vi "turn on off Keysight 9020A Correction Factor.vi"(8 "error in (no error)":errorcluster, 9 "Correction Applied?":bool, 10 "Target Correction Table":T1(ring), 11 "Keysight 9020A in":refnum<class "Keysight 9020A.lvclass">) -> (0 "error out":errorcluster, 3 "Keysight 9020A out":refnum<class "Keysight 9020A.lvclass">)   [LabVIEW 2023, in "Spectrum Analyzer.lvlib" / "Keysight 9020A.lvclass"]
uses:
  Keysight 9020A.lvclass
  Keysight 9020A.lvclass/Keysight 9020A.ctl
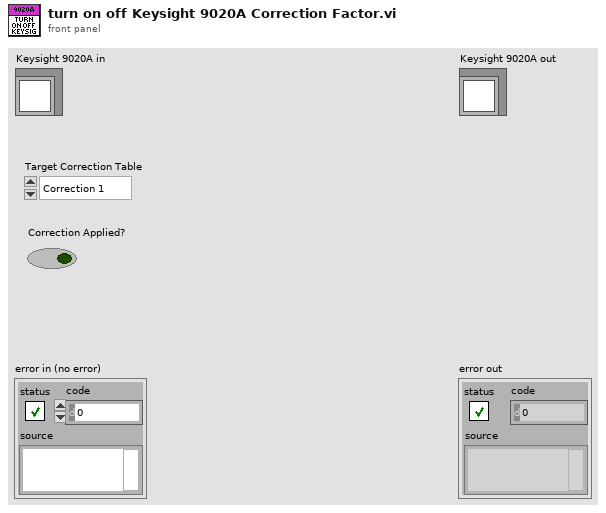
[diagram p1: front panel]
types:
  T1 = enum16{"Correction 1", "Correction 2", "Correction 3", "Correction 4", "Correction 5", "Correction 6", "Correction 7", "Correction 8"}
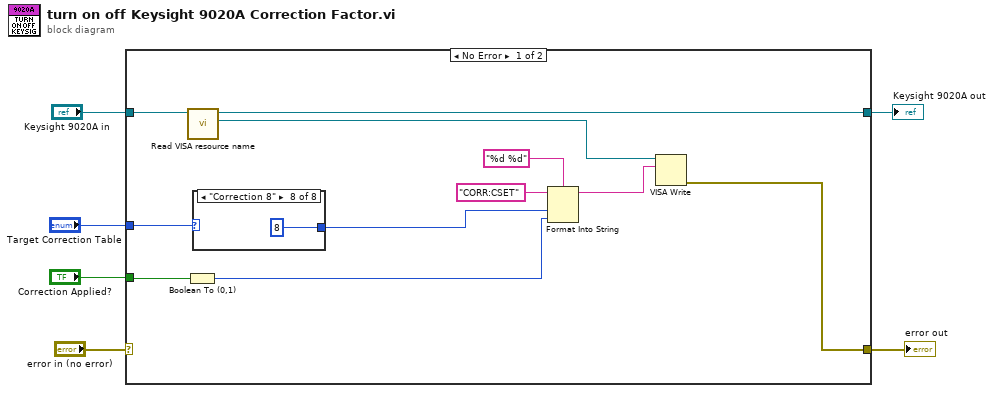
[diagram p0: block diagram]
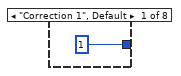
[diagram p2: hidden frame]
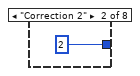
[diagram p3: hidden frame]
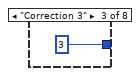
[diagram p4: hidden frame]
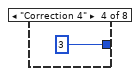
[diagram p5: hidden frame]
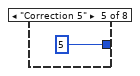
[diagram p6: hidden frame]
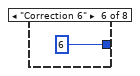
[diagram p7: hidden frame]
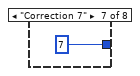
[diagram p8: hidden frame]
diagram:
  n1 = case shown="No Error" "error in (no error)" {
    selector: "error in (no error)" -> [_ w26]
    tunnel: "Keysight 9020A in" -> [w17 w27]
    tunnel: [w16 w27] -> w5
    tunnel: [w15 w26] -> w4
    tunnel: "Target Correction Table" -> [w10 _]
    tunnel: "Correction Applied?" -> [w9 _]
    frame No Error {
      n2 = Boolean To (0,1)(Boolean=w9) -> (0, 1=w8:i16)
      n3 = call "Read VISA resource name.vi"("Keysight 9020A in"=w17) -> ("VISA resource name"=w14:refnum<visa-resource-name>, "Keysight 9020A out"=w16:refnum<class "Keysight 9020A.lvclass">)  [unwired: 8 in, 1 out]
      n4 = case shown="\"Correction 8\"" w10 {
        tunnel: [1 2 3 3 5 6 7 8] -> w11
        frame "Correction 1", Default {
        }
        frame "Correction 2" {
        }
        frame "Correction 3" {
        }
        frame "Correction 4" {
        }
        frame "Correction 5" {
        }
        frame "Correction 6" {
        }
        frame "Correction 7" {
        }
        frame "Correction 8" {
        }
      }
      n5 = Format Into String(format string="%d %d", initial string="CORR:CSET", w11, w8) -> (resulting string=w7:string)  [unwired: 1 in, 1 out]
      n6 = VISA Write(VISA resource name=w14, write buffer=w7) -> (error out=w15:errorcluster)  [unwired: 1 in, 2 out]
    }
    frame Error {
    }
  }
  "error out" <- w4
  "Keysight 9020A out" <- w5
